vi "gRPC Server.vi"(8 "error in (no error)":errorcluster, 11 "CIFPlugin in":refnum<class "CAN_Reader_NIXNET_Plugin.lvclass">) -> (0 "error out":errorcluster, 3 "CIFPlugin out":refnum<class "CAN_Reader_NIXNET_Plugin.lvclass">)   [LabVIEW 2021, in "CAN_Reader_NIXNET_Plugin.lvclass"]
uses:
  CAN_Reader_NIXNET_Plugin.lvclass
  C:/Program Files/National Instruments/LabVIEW 2021/vi.lib/CIF Foundation/CIF Core/CIFCore/Class/CIFCorePlugin.lvclass
  CAN_Reader_NIXNET_Plugin.lvclass/CAN_Reader_NIXNET_Plugin.ctl
  <vilib>/xnet/xnet.llb/XNET Blink Modifier.ctl
  Grpc/CanReaderNixnet_server/RPC Messages/cif_common_Status.ctl
  Common/Typedef/Errors.ctl
  Grpc/CanReaderNixnet_server/RPC Messages/cif_can_reader_nixnet_XnetDevices.ctl
  Grpc/CanReaderNixnet_server/RPC Messages/cif_can_reader_nixnet_XnetDevice.ctl
  Grpc/CanReaderNixnet_server/RPC Messages/cif_can_reader_nixnet_Statistics.ctl
  <vilib>/CIF Foundation/CIF U8 Array Monitor gRPC/U8_Array_Monitor_gRPC/CIFU8ArrayMonitor_server/RPC Messages/cif_u8arraymonitor_SetEnableU8ArrayResponse.ctl
  <vilib>/CIF Foundation/CIF U8 Array Monitor gRPC/U8_Array_Monitor_gRPC/CIFU8ArrayMonitor_server/RPC Messages/cif_common_Status.ctl
  <vilib>/CIF Foundation/CIF U8 Array Monitor gRPC/U8_Array_Monitor_gRPC/CIFU8ArrayMonitor_server/RPC Messages/cif_u8arraymonitor_GetU8ArrayResponse.ctl
  <vilib>/CIF Foundation/CIF U8 Array Monitor gRPC/U8_Array_Monitor_gRPC/CIFU8ArrayMonitor_server/RPC Messages/cif_u8arraymonitor_U8Arrays.ctl
  <vilib>/CIF Foundation/CIF U8 Array Monitor gRPC/U8_Array_Monitor_gRPC/CIFU8ArrayMonitor_server/RPC Messages/cif_u8arraymonitor_U8Array.ctl
  Grpc/CanReaderNixnet_server/RPC Messages/Get cif_can_reader_nixnet_InterfaceBlink.vi
  Grpc/CanReaderNixnet_server/RPC Messages/Set cif_common_Status.vi
  Grpc/CanReaderNixnet_server/RPC Messages/Get cif_can_reader_nixnet_RefreshDevices.vi
  Grpc/CanReaderNixnet_server/RPC Messages/Set cif_can_reader_nixnet_XnetDevices.vi
  Grpc/CanReaderNixnet_server/RPC Messages/Set cif_can_reader_nixnet_Statistics.vi
  Grpc/CanReaderNixnet_server/RPC Messages/Get cif_common_Empty.vi
  <vilib>/CIF Foundation/CIF U8 Array Monitor gRPC/U8_Array_Monitor_gRPC/CIFU8ArrayMonitor_server/RPC Messages/Get cif_u8arraymonitor_SetEnableU8ArrayRequest.vi
  <vilib>/CIF Foundation/CIF U8 Array Monitor gRPC/U8_Array_Monitor_gRPC/CIFU8ArrayMonitor_server/RPC Messages/Set cif_u8arraymonitor_SetEnableU8ArrayResponse.vi
  <vilib>/CIF Foundation/CIF U8 Array Monitor gRPC/U8_Array_Monitor_gRPC/CIFU8ArrayMonitor_server/RPC Messages/Get cif_u8arraymonitor_GetU8ArrayRequest.vi
  <vilib>/CIF Foundation/CIF U8 Array Monitor gRPC/U8_Array_Monitor_gRPC/CIFU8ArrayMonitor_server/RPC Messages/Set cif_u8arraymonitor_GetU8ArrayResponse.vi
  Grpc/CanReaderNixnet_server/RPC Messages/Get cif_can_reader_nixnet_InterfaceBlink.vi/2ed25e12-861d-4677-8ead-ace2906b2041.vi
  Grpc/CanReaderNixnet_server/RPC Messages/FlatToRichcif_can_reader_nixnet_InterfaceBlink.vi
  Grpc/CanReaderNixnet_server/RPC Messages/Set cif_common_Status.vi/dcc74a39-081a-4bdd-860b-8ed792803c96.vi
  Grpc/CanReaderNixnet_server/RPC Messages/RichToFlatcif_common_Status.vi
  Grpc/CanReaderNixnet_server/RPC Messages/Get cif_can_reader_nixnet_RefreshDevices.vi/2ed25e12-861d-4677-8ead-ace2906b2041.vi
  Grpc/CanReaderNixnet_server/RPC Messages/FlatToRichcif_can_reader_nixnet_RefreshDevices.vi
  Grpc/CanReaderNixnet_server/RPC Messages/Set cif_can_reader_nixnet_XnetDevices.vi/dcc74a39-081a-4bdd-860b-8ed792803c96.vi
  Grpc/CanReaderNixnet_server/RPC Messages/RichToFlatcif_can_reader_nixnet_XnetDevices.vi
  Grpc/CanReaderNixnet_server/RPC Messages/Set cif_can_reader_nixnet_Statistics.vi/dcc74a39-081a-4bdd-860b-8ed792803c96.vi
  Grpc/CanReaderNixnet_server/RPC Messages/RichToFlatcif_can_reader_nixnet_Statistics.vi
  Grpc/CanReaderNixnet_server/RPC Messages/Get cif_common_Empty.vi/2ed25e12-861d-4677-8ead-ace2906b2041.vi
  Grpc/CanReaderNixnet_server/RPC Messages/FlatToRichcif_common_Empty.vi
  <vilib>/CIF Foundation/CIF U8 Array Monitor gRPC/U8_Array_Monitor_gRPC/CIFU8ArrayMonitor_server/RPC Messages/Get cif_u8arraymonitor_SetEnableU8ArrayRequest.vi/2ed25e12-861d-4677-8ead-ace2906b2041.vi
  <vilib>/CIF Foundation/CIF U8 Array Monitor gRPC/U8_Array_Monitor_gRPC/CIFU8ArrayMonitor_server/RPC Messages/FlatToRichcif_u8arraymonitor_SetEnableU8ArrayRequest.vi
  <vilib>/CIF Foundation/CIF U8 Array Monitor gRPC/U8_Array_Monitor_gRPC/CIFU8ArrayMonitor_server/RPC Messages/Set cif_u8arraymonitor_SetEnableU8ArrayResponse.vi/dcc74a39-081a-4bdd-860b-8ed792803c96.vi
  <vilib>/CIF Foundation/CIF U8 Array Monitor gRPC/U8_Array_Monitor_gRPC/CIFU8ArrayMonitor_server/RPC Messages/RichToFlatcif_u8arraymonitor_SetEnableU8ArrayResponse.vi
  <vilib>/CIF Foundation/CIF U8 Array Monitor gRPC/U8_Array_Monitor_gRPC/CIFU8ArrayMonitor_server/RPC Messages/Get cif_u8arraymonitor_GetU8ArrayRequest.vi/2ed25e12-861d-4677-8ead-ace2906b2041.vi
  <vilib>/CIF Foundation/CIF U8 Array Monitor gRPC/U8_Array_Monitor_gRPC/CIFU8ArrayMonitor_server/RPC Messages/FlatToRichcif_u8arraymonitor_GetU8ArrayRequest.vi
  <vilib>/CIF Foundation/CIF U8 Array Monitor gRPC/U8_Array_Monitor_gRPC/CIFU8ArrayMonitor_server/RPC Messages/Set cif_u8arraymonitor_GetU8ArrayResponse.vi/dcc74a39-081a-4bdd-860b-8ed792803c96.vi
  <vilib>/CIF Foundation/CIF U8 Array Monitor gRPC/U8_Array_Monitor_gRPC/CIFU8ArrayMonitor_server/RPC Messages/RichToFlatcif_u8arraymonitor_GetU8ArrayResponse.vi
  <vilib>/gRPC/LabVIEW gRPC Library/Shared/TranslateGrpcError.vi
  Grpc/CanReaderNixnet_server/RPC Messages/RichToFlatcif_can_reader_nixnet_XnetDevice.vi
  <vilib>/CIF Foundation/CIF U8 Array Monitor gRPC/U8_Array_Monitor_gRPC/CIFU8ArrayMonitor_server/RPC Messages/RichToFlatcif_common_Status.vi
  <vilib>/CIF Foundation/CIF U8 Array Monitor gRPC/U8_Array_Monitor_gRPC/CIFU8ArrayMonitor_server/RPC Messages/RichToFlatcif_u8arraymonitor_U8Arrays.vi
  <vilib>/CIF Foundation/CIF U8 Array Monitor gRPC/U8_Array_Monitor_gRPC/CIFU8ArrayMonitor_server/RPC Messages/RichToFlatcif_u8arraymonitor_U8Array.vi
  <vilib>/gRPC/LabVIEW gRPC Library/Server API/Server/Get Server DLL Path.vi
  <vilib>/Utility/error.llb/Error Cluster From Error Code.vi
  Common/SubVIs/Add Error Core.vi
  <vilib>/gRPC/LabVIEW gRPC Library/Server API/Message Requests/Complete Call.vi
  <vilib>/CIF Foundation/CIF Core/CIFCore/Class/CIFCorePlugin.lvclass
  Grpc/CanReaderNixnet_server/CanReaderNixnet_server.lvlib
  Grpc/CanReaderNixnet_server/RPC Service/CanReaderNixnet/CanReaderNixnet.lvclass
  <vilib>/CIF Foundation/CIF U8 Array Monitor gRPC/U8_Array_Monitor_gRPC/CIFU8ArrayMonitor_server/RPC Service/U8ArrayMonitor/U8ArrayMonitor.lvclass
  <vilib>/CIF Foundation/CIF U8 Array Monitor gRPC/U8_Array_Monitor_gRPC/CIFU8ArrayMonitorUtilities/CIFU8ArrayMonitorUtilities.lvlib
  <vilib>/CIF Foundation/CIF U8 Array Monitor gRPC/U8_Array_Monitor_gRPC/CIFU8ArrayMonitor_server/CIFU8ArrayMonitor_server.lvlib
  <vilib>/CIF Foundation/CIF XNET CAN RW/XNET CAN RW.lvclass
  Common/CAN_Reader_NIXNET_Common.lvlib
  Grpc/CanReaderNixnet_server/RPC Messages/cif_can_reader_nixnet_CommState.ctl
  Grpc/CanReaderNixnet_server/RPC Messages/cif_can_reader_nixnet_LastError.ctl
  Grpc/CanReaderNixnet_server/RPC Messages/cif_can_reader_nixnet_GetCANStatusResponse.ctl
  D:/dev/Plugins/CAN_Reader_NIXNET/Class/CAN_Reader_NIXNET_Plugin.lvclass
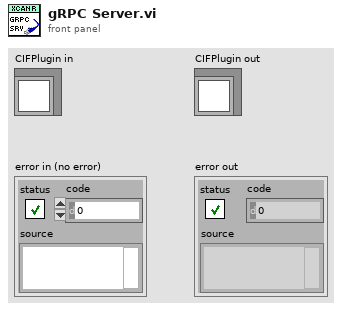
[diagram p1: front panel]
types:
  T1 = typedef "CanReaderNixnet_server.lvlib/cif_common_Status.ctl" = cluster{"code":i32, "message":string}
  T2 = typedef "CAN_Reader_NIXNET_Common.lvlib/Errors.ctl" = enum16{"Invalid Interface"}
  T3 = typedef "CanReaderNixnet_server.lvlib/cif_can_reader_nixnet_XnetDevices.ctl" = cluster{"devices":T4[]}
  T4 = typedef "CanReaderNixnet_server.lvlib/cif_can_reader_nixnet_XnetDevice.ctl" = cluster{"interface":string, "slot":u32, "device_id":string}
  T5 = typedef "CanReaderNixnet_server.lvlib/cif_can_reader_nixnet_Statistics.ctl" = cluster{"iterations":u64, "read_timeouts":u64, "read_frames":u64, "filtered_frames":u64}
  T6 = typedef "CIFU8ArrayMonitor_server.lvlib/cif_u8arraymonitor_SetEnableU8ArrayResponse.ctl" = cluster{"status":T7}
  T7 = typedef "CIFU8ArrayMonitor_server.lvlib/cif_common_Status.ctl" = cluster{"code":i32, "message":string}
  T8 = typedef "CIFU8ArrayMonitor_server.lvlib/cif_u8arraymonitor_GetU8ArrayResponse.ctl" = cluster{"u8arrays":T9}
  T9 = typedef "CIFU8ArrayMonitor_server.lvlib/cif_u8arraymonitor_U8Arrays.ctl" = cluster{"u8_array":T10[], "valid":bool}
  T10 = typedef "CIFU8ArrayMonitor_server.lvlib/cif_u8arraymonitor_U8Array.ctl" = cluster{"u8_array":u8[], "timestamp":i64}
  T11 = typedef "CanReaderNixnet_server.lvlib/cif_can_reader_nixnet_GetCANStatusResponse.ctl" = cluster{"comm_state":T12, "last_error":T13, "rx_error_ctr":u32, "tx_error_crt":u32}
  T12 = typedef "CanReaderNixnet_server.lvlib/cif_can_reader_nixnet_CommState.ctl" = enum32{"COMMSTATE_ERROR_ACTIVE", "COMMSTATE_ERROR_PASSIVE", "COMMSTATE_BUS_OFF"}
  T13 = typedef "CanReaderNixnet_server.lvlib/cif_can_reader_nixnet_LastError.ctl" = enum32{"LASTERROR_NONE", "LASTERROR_STUFF", "LASTERROR_FORM", "LASTERROR_ACK", "LASTERROR_BIT1", "LASTERROR_BIT0", "LASTERROR_CRC", "LASTERROR_UNKNOWN"}
  T14 = typedef "XNET CAN RW.lvclass/XNET Devices.ctl" = cluster{"ID":string, "Slot":u32, "Interfaces":string[]}
  T15 = typedef "XNET Blink Modifier.ctl" = u32
  T16 = typedef "grpc-lvsupport-release.lvlib/grpcId.ctl" = u64
  T17 = typedef "CanReaderNixnet_server.lvlib/cif_can_reader_nixnet_InterfaceBlink.ctl" = cluster{"blink":bool}
  T18 = typedef "CAN_Reader_NIXNET_Common.lvlib/Configuration.ctl" = cluster{"Common":T19, "RX Interface":string, "Port Configuration":T21, "Timeout (ms)":i32, "Frames to read":i32, "Filter":T24}
  T19 = typedef "CIFCoreCommon.lvlib/Common Plugin Configuration.ctl" = cluster{"Period (s)":dbl, "Offset (us)":i32, "Priority":i32, "Processor":i32, "External Clock":T20}
  T20 = typedef "CIFCoreCommon.lvlib/External Clock Config.ctl" = cluster{"ClockID":u8, "Clock Name":string, "Publish Clock":bool, "Convert Data Timestamps":bool, "Plugin Timing Source":bool}
  T21 = typedef "CAN_RW_CORE.lvclass/CAN Port Configuration.ctl" = cluster{"Mode":T22, "Baud Rate":u64, "Temination On":bool, "Subordinate":bool, "Echo TX":bool, "FD Config":T23}
  T22 = typedef "CAN_RW_CORE.lvclass/CAN Mode.ctl" = enum16{"CAN 2.0", "CAN FD"}
  T23 = typedef "CAN_RW_CORE.lvclass/FD Config.ctl" = cluster{"FD Baud Rate":u64, "ISO Mode":bool, "BRS Enabled":bool}
  T24 = typedef "CAN_RW_CORE.lvclass/CAN Filter.ctl" = cluster{"Allow List (ID)":u32[], "Deny List (ID)":u32[]}
  T25 = typedef "CanReaderNixnet_server.lvlib/cif_can_reader_nixnet_RefreshDevices.ctl" = cluster{"refresh_device_list":bool}
  T26 = typedef "CIFU8ArrayMonitor_server.lvlib/cif_u8arraymonitor_SetEnableU8ArrayRequest.ctl" = cluster{"enable_u8_array":bool, "history_depth":u32}
  T27 = typedef "CIFU8ArrayMonitorUtilities.lvlib/gRPC to Main Data.ctl" = cluster{"Enable U8 Array":bool, "History Depth":u32}
  T28 = typedef "CIFU8ArrayMonitorUtilities.lvlib/CIF U8 Array DVR.ctl" = refnum<data-value>
  T29 = typedef "CIFU8ArrayMonitor_client.lvlib/cif_u8arraymonitor_U8Arrays.ctl" = cluster{"u8_array":T30[], "valid":bool}
  T30 = typedef "CIFU8ArrayMonitor_client.lvlib/cif_u8arraymonitor_U8Array.ctl" = cluster{"u8_array":u8[], "timestamp":i64}
  T31 = typedef "CAN_RW_CORE.lvclass/Communication State.ctl" = enum16{"Error Active", "Error Passive", "Bus Off"}
  T32 = typedef "CAN_RW_CORE.lvclass/Last Error.ctl" = enum16{"None", "Stuff", "Form", "Ack", "Bit1", "Bit0", "CRC", "Unknown"}
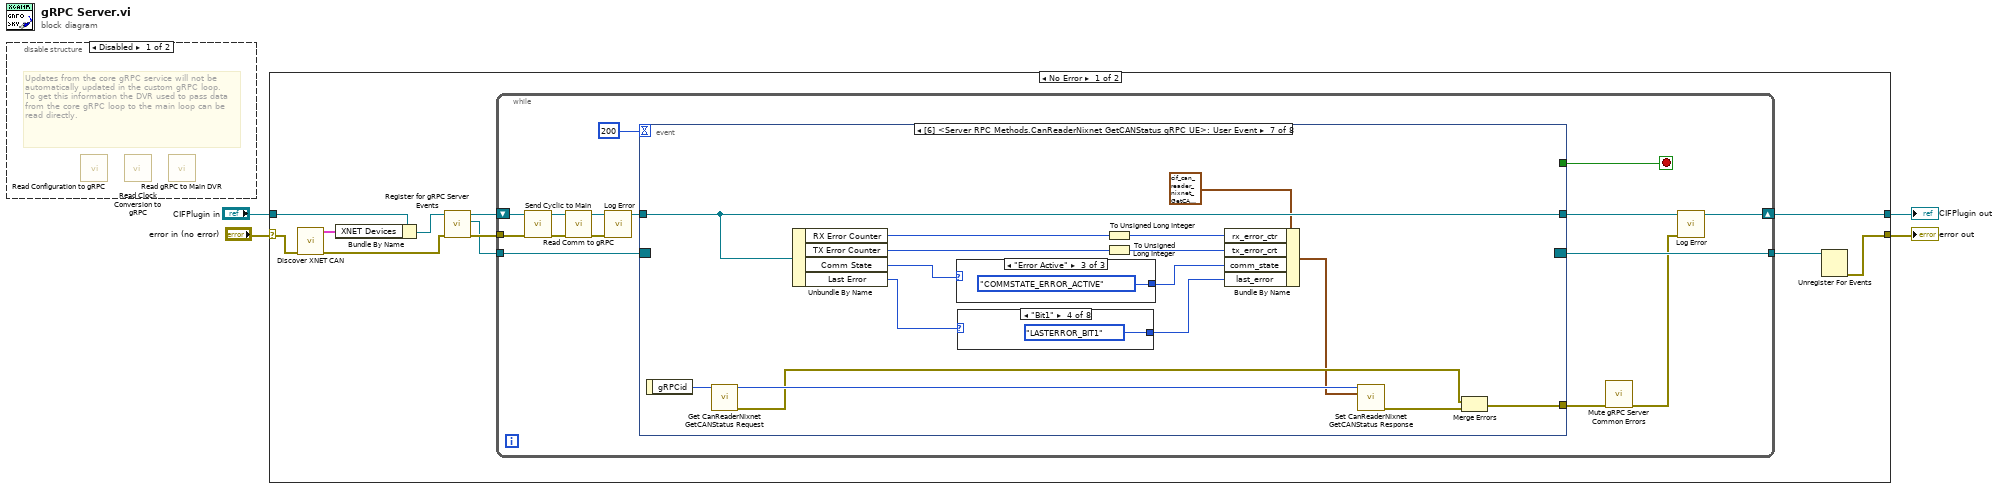
[diagram p0: block diagram]
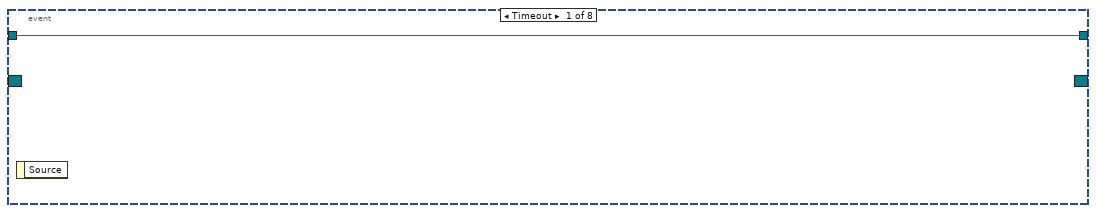
[diagram p3: hidden frame]
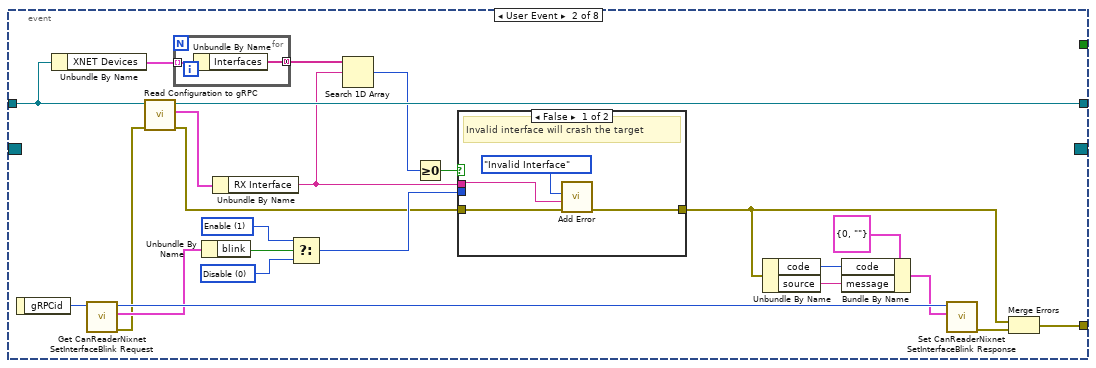
[diagram p4: hidden frame]
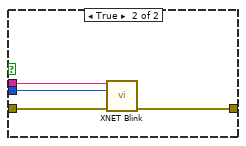
[diagram p5: hidden frame]
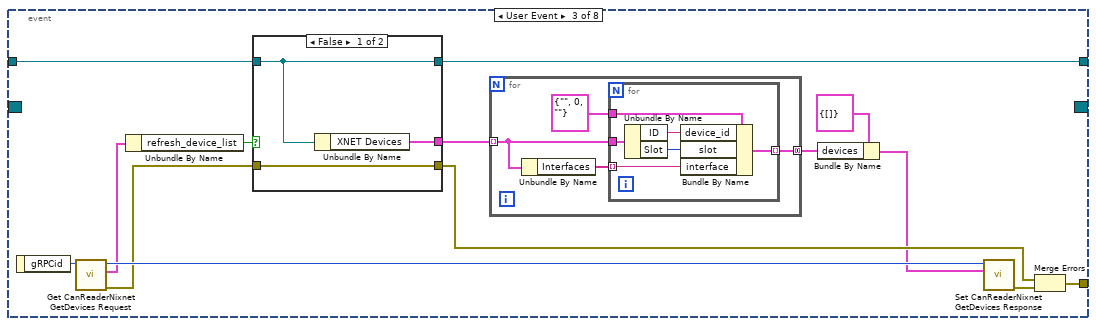
[diagram p6: hidden frame]
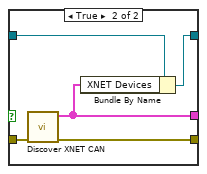
[diagram p7: hidden frame]
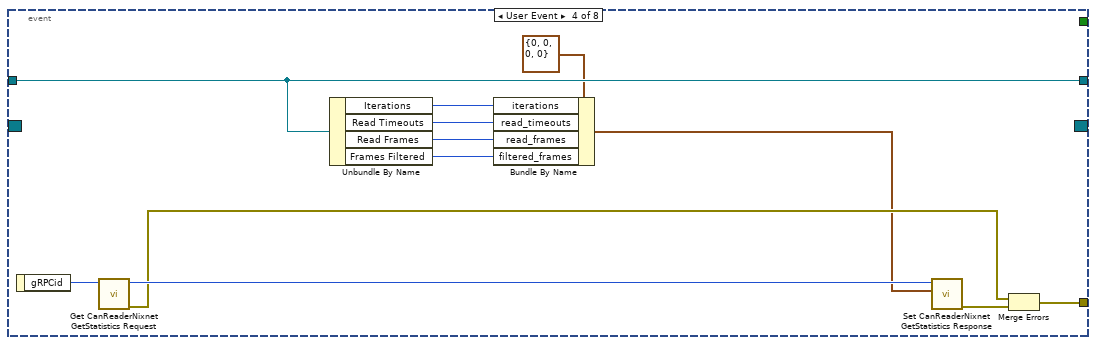
[diagram p8: hidden frame]
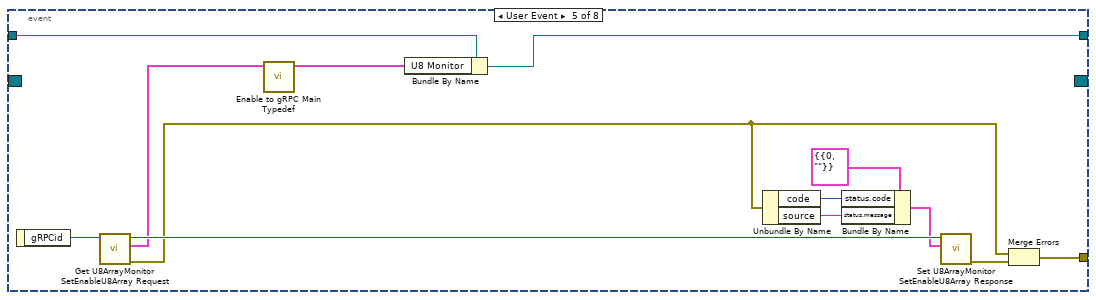
[diagram p9: hidden frame]
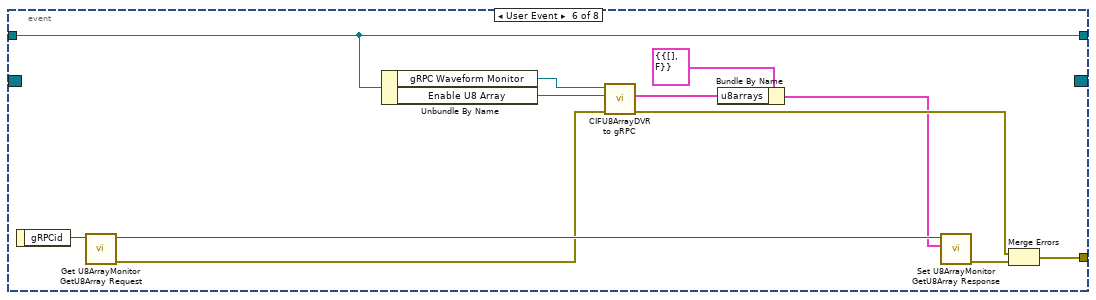
[diagram p10: hidden frame]
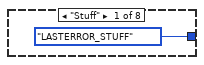
[diagram p11: hidden frame]
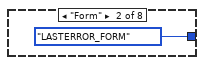
[diagram p12: hidden frame]
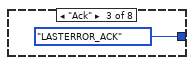
[diagram p13: hidden frame]
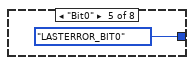
[diagram p14: hidden frame]
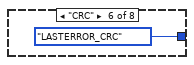
[diagram p15: hidden frame]
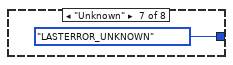
[diagram p16: hidden frame]
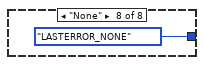
[diagram p17: hidden frame]
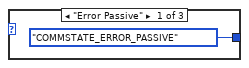
[diagram p18: hidden frame]
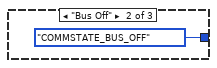
[diagram p19: hidden frame]
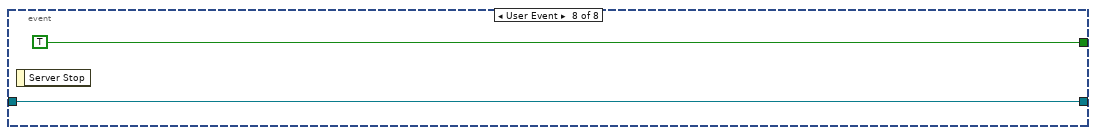
[diagram p20: hidden frame]
diagram:
  n1 = disable-structure shown="Disabled" {
    frame Disabled {
      # "Updates from the core gRPC service will not be automatically updated in the custom gRPC loop.  To get this information the DVR used to pass data from the core gRPC loop to the main loop can be read directly."
      n2 = call "Read Configuration to gRPC.vi"() -> ()  [unwired: 9 in, 3 out]
      n3 = call <vilib>:"Read Clock Conversion to gRPC.vi"() -> ()  [unwired: 9 in, 3 out]
      n4 = call <vilib>:"Read gRPC to Main DVR.vi"() -> ()  [unwired: 9 in, 3 out]
    }
    frame Enabled {
    }
  }
  n5 = case shown="No Error" "error in (no error)" {
    selector: "error in (no error)" -> [w7 w164]
    tunnel: "CIFPlugin in" -> [w9 w165]
    tunnel: [w14 w165] -> w3
    tunnel: [w11 w164] -> w4
    frame No Error {
      n6 = call <vilib>:"Discover XNET CAN.vi"("error in (no error)"=w7) -> ("error out"=w6:errorcluster, "XNET Devices"=w10:T14[])  [unwired: 9 in]
      n7 = Bundle By Name(cluster=w9, "XNET Devices"=w10) -> (w8:refnum<class "CAN_Reader_NIXNET_Plugin.lvclass">)
      n8 = call "Register for gRPC Server Events.vi"("error in (no error)"=w6, "CIFPlugin in"=w8) -> ("error out"=w13:errorcluster, "Event Registration Refnum"=w5:refnum<event-registration>, "CIFPlugin out"=w12:refnum<class "CAN_Reader_NIXNET_Plugin.lvclass">)  [unwired: 7 in]
      n9 = while {
        tunnel: w13 -> [w23]
        tunnel: [w28] -> w15
        shift-right: [w26] -> w14
        shift-left: w12 -> [w24]
        tunnel: w5 -> [w18]
        stop <- w29 stop-if-true
        n10 = call "Send Cyclic to Main.vi"("error in (no error)"=w23, "CIFPlugin in"=w24) -> ("error out"=w21:errorcluster, "CIFPlugin out"=w22:refnum<class "CAN_Reader_NIXNET_Plugin.lvclass">)  [unwired: 8 in]
        n11 = call "Read Comm to gRPC.vi"("error in (no error)"=w21, "CIFPlugin in"=w22) -> ("error out"=w19:errorcluster, "CIFPlugin out"=w20:refnum<class "CAN_Reader_NIXNET_Plugin.lvclass">)  [unwired: 8 in]
        n12 = call <vilib>:"Log Error.vi"("error in (no error)"=w19, "CIFCorePlugin in"=w20) -> ("CIFCorePlugin out"=w25:refnum<class "CAN_Reader_NIXNET_Plugin.lvclass">)  [unwired: 8 in, 1 out]
        n13 = event shown="[6] <Server RPC Methods.CanReaderNixnet GetCANStatus gRPC UE>: User Event" {
          selector: w18 -> [_ _ _ _ _ _ _ _]
          dyn-events: [_ _ _ _ _ _ _ _] -> w28
          timeout: 200 -> [_ _ _ _ _ _ _ _]
          tunnel: w25 -> [w31 w36 w73 w108 w119 w130 w142 w162]
          tunnel: [_ w53 w79 w109 w120 w134 w139 _] -> w17
          tunnel: [w31 w38 w70 w108 w118 w130 w142 w162] -> w27
          tunnel: [_ _ _ _ _ _ _ TRUE] -> w29
          event Timeout {
            n14 = event-data() -> ()  [unwired: 1 in, 1 out]
          }
          event User Event {
            w44 = T15 1 items=["Disable", "Enable"] ("modifier")
            w45 = T15 0 items=["Disable", "Enable"] ("modifier")
            n15 = event-data() -> ("gRPCid"=w48:T16)  [unwired: 1 in]
            n16 = Unbundle By Name(w36) -> ("XNET Devices"=w37:T14[])
            n17 = call "Get CanReaderNixnet SetInterfaceBlink Request.vi"("gRPCid"=w48) -> ("error out"=w40:errorcluster, "Message Data"=w47:T17, "gRPCid out"=w51:T16)  [unwired: 8 in]
            n18 = call "Read Configuration to gRPC.vi"("error in (no error)"=w40, "CIFPlugin in"=w36) -> ("error out"=w39:errorcluster, "Configuration"=w41:T18, "CIFPlugin out"=w38:refnum<class "CAN_Reader_NIXNET_Plugin.lvclass">)  [unwired: 7 in]
            n19 = for {
              tunnel: w37 -> [w57] mode=indexing
              tunnel: [w56] -> w35 mode=concatenating
              n20 = Unbundle By Name(w57) -> ("Interfaces"=w56:string[])
            }
            n21 = Unbundle By Name(w47) -> ("blink"=w46:bool)
            n22 = Unbundle By Name(w41) -> ("RX Interface"=w34:string)
            n23 = Select(t=w44, s=w46, f=w45) -> (s? t:f=w42:T15)
            n24 = Search 1D Array(1D array=w35, element=w34) -> (index of element=w33:i32)  [unwired: 1 in]
            n25 = Greater Or Equal To 0?(x=w33) -> (x >= 0?=w32:bool)
            n26 = case shown="False" w32 {
              tunnel: w34 -> [w59 w65]
              tunnel: w39 -> [w61 w64]
              tunnel: [w60 w63] -> w43
              tunnel: w42 -> [_ w62]
              frame False {
                # "Invalid interface will crash the target"
                n27 = call "Add Error.vi"("error in (no error)"=w61, "String to Append"=w59, "Error"=Errors."Invalid Interface") -> ("error out"=w60:errorcluster)  [unwired: 8 in]
              }
              frame True {
                n28 = call <vilib>:"XNET Blink.vi"("interface in"=w65, "modifier"=w62, "error in (no error)"=w64) -> ("error out"=w63:errorcluster)  [unwired: 11 in, 1 out]
              }
            }
            n29 = Unbundle By Name(w43) -> ("code"=w55:i32, "source"=w54:string)
            n30 = Bundle By Name(cluster=T1 {"code"=0, "message"=""} ("Status"), "code"=w55, "message"=w54) -> (w49:T1)
            n31 = call "Set CanReaderNixnet SetInterfaceBlink Response.vi"("Message Data"=w49, "gRPCid in"=w51) -> ("error out"=w50:errorcluster)  [unwired: 9 in]
            n32 = Merge Errors(w43, w50) -> (w53:errorcluster)
          }
          event User Event {
            n33 = event-data() -> ("gRPCid"=w76:T16)  [unwired: 1 in]
            n34 = call "Get CanReaderNixnet GetDevices Request.vi"("gRPCid"=w76) -> ("error out"=w72:errorcluster, "Message Data"=w75:T25, "gRPCid out"=w78:T16)  [unwired: 8 in]
            n35 = Unbundle By Name(w75) -> ("refresh_device_list"=w74:bool)
            n36 = case shown="False" w74 {
              tunnel: w73 -> [w91 w97]
              tunnel: w72 -> [w92 w96]
              tunnel: [w92 w95] -> w71
              tunnel: [w91 w94] -> w70
              tunnel: [w90 w93] -> w66
              frame False {
                n37 = Unbundle By Name(w91) -> ("XNET Devices"=w90:T14[])
              }
              frame True {
                n38 = call <vilib>:"Discover XNET CAN.vi"("error in (no error)"=w96) -> ("error out"=w95:errorcluster, "XNET Devices"=w93:T14[])  [unwired: 9 in]
                n39 = Bundle By Name(cluster=w97, "XNET Devices"=w93) -> (w94:refnum<class "CAN_Reader_NIXNET_Plugin.lvclass">)
              }
            }
            n40 = for {
              tunnel: w66 -> [w82] mode=indexing
              tunnel: [w81] -> w67 mode=concatenating
              n41 = Unbundle By Name(w82) -> ("Interfaces"=w83:string[])
              n42 = for {
                tunnel: w83 -> [w86] mode=indexing
                tunnel: w82 -> [w89]
                tunnel: T4 {"interface"="", "slot"=0, "device_id"=""} ("cif_can_reader_nixnet_XnetDevice") -> [w88]
                tunnel: [w84] -> w81 mode=indexing
                n43 = Unbundle By Name(w89) -> ("ID"=w87:string, "Slot"=w85:u32)
                n44 = Bundle By Name(cluster=w88, "device_id"=w87, "slot"=w85, "interface"=w86) -> (w84:T4)
              }
            }
            n45 = Bundle By Name(cluster=T3 {"devices"=[]} ("Message Data"), "devices"=w67) -> (w69:T3)
            n46 = call "Set CanReaderNixnet GetDevices Response.vi"("Message Data"=w69, "gRPCid in"=w78) -> ("error out"=w77:errorcluster)  [unwired: 9 in]
            n47 = Merge Errors(w71, w77) -> (w79:errorcluster)
          }
          event User Event {
            n48 = event-data() -> ("gRPCid"=w106:T16)  [unwired: 1 in]
            n49 = call "Get CanReaderNixnet GetStatistics Request.vi"("gRPCid"=w106) -> ("error out"=w103:errorcluster, "gRPCid out"=w105:T16)  [unwired: 8 in, 1 out]
            n50 = Unbundle By Name(w108) -> ("Iterations"=w107:u64, "Read Timeouts"=w98:u64, "Read Frames"=w99:u64, "Frames Filtered"=w100:u64)
            n51 = Bundle By Name(cluster=T5 {"iterations"=0, "read_timeouts"=0, "read_frames"=0, "filtered_frames"=0} ("Statistics"), "iterations"=w107, "read_timeouts"=w98, "read_frames"=w99, "filtered_frames"=w100) -> (w102:T5)
            n52 = call "Set CanReaderNixnet GetStatistics Response.vi"("Message Data"=w102, "gRPCid in"=w105) -> ("error out"=w104:errorcluster)  [unwired: 9 in]
            n53 = Merge Errors(w103, w104) -> (w109:errorcluster)
          }
          event User Event {
            n54 = event-data() -> ("gRPCid"=w115:T16)  [unwired: 1 in]
            n55 = call <vilib>:"Get U8ArrayMonitor SetEnableU8Array Request.vi"("gRPCid"=w115) -> ("error out"=w114:errorcluster, "Message Data"=w116:T26, "gRPCid out"=w117:T16)  [unwired: 8 in]
            n56 = call <vilib>:"Enable to gRPC Main Typedef.vi"("U8ArrayEnable"=w116) -> ("gRPC to Main Data"=w112:T27)  [unwired: 10 in]
            n57 = Bundle By Name(cluster=w119, "U8 Monitor"=w112) -> (w118:refnum<class "CAN_Reader_NIXNET_Plugin.lvclass">)
            n58 = Unbundle By Name(w114) -> ("code"=w122:i32, "source"=w121:string)
            n59 = Bundle By Name(cluster=T6 {"status"={"code"=0, "message"=""}} ("Message Data"), "status.code"=w122, "status.message"=w121) -> (w111:T6)
            n60 = call <vilib>:"Set U8ArrayMonitor SetEnableU8Array Response.vi"("Message Data"=w111, "gRPCid in"=w117) -> ("error out"=w113:errorcluster)  [unwired: 9 in]
            n61 = Merge Errors(w114, w113) -> (w120:errorcluster)
          }
          event User Event {
            n62 = event-data() -> ("gRPCid"=w132:T16)  [unwired: 1 in]
            n63 = call <vilib>:"Get U8ArrayMonitor GetU8Array Request.vi"("gRPCid"=w132) -> ("error out"=w129:errorcluster, "gRPCid out"=w133:T16)  [unwired: 8 in, 1 out]
            n64 = Unbundle By Name(w130) -> ("gRPC Waveform Monitor"=w126:T28, "Enable U8 Array"=w127:bool)
            n65 = call <vilib>:"CIFU8ArrayDVR to gRPC .vi"("error in (no error)"=w129, "gRPC Waveform Enabled"=w127, "gRPC Waveform Monitor in"=w126) -> ("error out"=w128:errorcluster, "U8 Array Monitor"=w124:T29)  [unwired: 6 in, 1 out]
            n66 = Bundle By Name(cluster=T8 {"u8arrays"={"u8_array"=[], "valid"=FALSE}} ("Message Data"), "u8arrays"=w124) -> (w123:T8)
            n67 = call <vilib>:"Set U8ArrayMonitor GetU8Array Response.vi"("Message Data"=w123, "gRPCid in"=w133) -> ("error out"=w131:errorcluster)  [unwired: 9 in]
            n68 = Merge Errors(w128, w131) -> (w134:errorcluster)
          }
          event User Event {
            n69 = event-data() -> ("gRPCid"=w141:T16)  [unwired: 1 in]
            n70 = call "Get CanReaderNixnet GetCANStatus Request.vi"("gRPCid"=w141) -> ("error out"=w137:errorcluster, "gRPCid out"=w138:T16)  [unwired: 8 in, 1 out]
            n71 = Unbundle By Name(w142) -> ("RX Error Counter"=w143:u8, "TX Error Counter"=w144:u8, "Comm State"=w147:T31, "Last Error"=w149:T32)
            n72 = case shown="\"Error Active\"" w147 {
              tunnel: [cif_can_reader_nixnet_CommState."COMMSTATE_ERROR_PASSIVE" ("comm_state") cif_can_reader_nixnet_CommState."COMMSTATE_BUS_OFF" ("comm_state") cif_can_reader_nixnet_CommState."COMMSTATE_ERROR_ACTIVE" ("comm_state")] -> w148
              frame "Error Passive" {
              }
              frame "Bus Off" {
              }
              frame "Error Active" {
              }
            }
            n73 = case shown="\"Bit1\"" w149 {
              tunnel: [cif_can_reader_nixnet_LastError."LASTERROR_STUFF" ("last_error") cif_can_reader_nixnet_LastError."LASTERROR_FORM" ("last_error") cif_can_reader_nixnet_LastError."LASTERROR_ACK" ("last_error") cif_can_reader_nixnet_LastError."LASTERROR_BIT1" ("last_error") cif_can_reader_nixnet_LastError."LASTERROR_BIT0" ("last_error") cif_can_reader_nixnet_LastError."LASTERROR_CRC" ("last_error") cif_can_reader_nixnet_LastError."LASTERROR_UNKNOWN" ("last_error") cif_can_reader_nixnet_LastError."LASTERROR_NONE" ("last_error")] -> w150
              frame "Stuff" {
              }
              frame "Form" {
              }
              frame "Ack" {
              }
              frame "Bit1" {
              }
              frame "Bit0" {
              }
              frame "CRC" {
              }
              frame "Unknown" {
              }
              frame "None" {
              }
            }
            n74 = To Unsigned Long Integer(number=w143) -> (unsigned 32bit integer=w146:u32)
            n75 = To Unsigned Long Integer(number=w144) -> (unsigned 32bit integer=w145:u32)
            n76 = Bundle By Name(cluster=T11 {"comm_state"=enum."COMMSTATE_ERROR_ACTIVE", "last_error"=enum."LASTERROR_NONE", "rx_error_ctr"=0, "tx_error_crt"=0} ("Message Data"), "rx_error_ctr"=w146, "tx_error_crt"=w145, "comm_state"=w148, "last_error"=w150) -> (w135:T11)
            n77 = call "Set CanReaderNixnet GetCANStatus Response.vi"("Message Data"=w135, "gRPCid in"=w138) -> ("error out"=w140:errorcluster)  [unwired: 9 in]
            n78 = Merge Errors(w137, w140) -> (w139:errorcluster)
          }
          event User Event {
            n79 = event-data() -> ()  [unwired: 1 in, 1 out]
          }
        }
        n80 = call <vilib>:"Mute gRPC Server Common Errors.vi"("error in (no error)"=w17) -> ("error out"=w16:errorcluster)  [unwired: 10 in]
        n81 = call <vilib>:"Log Error.vi"("error in (no error)"=w16, "CIFCorePlugin in"=w27) -> ("CIFCorePlugin out"=w26:refnum<class "CAN_Reader_NIXNET_Plugin.lvclass">)  [unwired: 8 in, 1 out]
      }
      n82 = Unregister For Events(event registration refnum=w15) -> (error out=w11:errorcluster)  [unwired: 1 in]
    }
    frame Error {
    }
  }
  "error out" <- w4
  "CIFPlugin out" <- w3
